vi "libssh2_session_get_timeout.vi"(8 "error in (no error)":errorcluster, 11 "session":T1) -> (0 "error out":errorcluster, 2 "timeout in ms":i32)   [LabVIEW 2017, in "libssh2.lvlib"]
doc: "Get the timeout for blocking functions on a session. A value of zero indicates no timeout."
uses:
  libssh2.lvlib
  Session Refnum.ctl
  Not A Session.vi
  <vilib>/Utility/error.llb/Error Cluster From Error Code.vi
  Global Settings.vi
  Read Session Refnum.vi
  <vilib>/Utility/semaphor.llb/Acquire Semaphore.vi
  <vilib>/Utility/semaphor.llb/Release Semaphore.vi
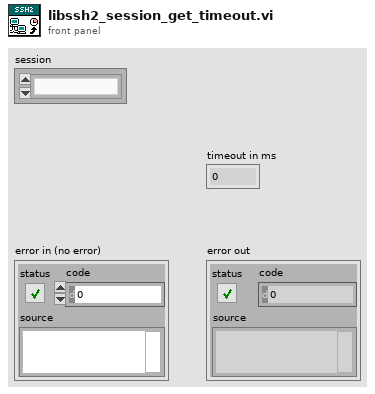
[diagram p1: front panel]
types:
  T1 = typedef "libssh2.lvlib/Session Refnum.ctl" = refnum<k1>
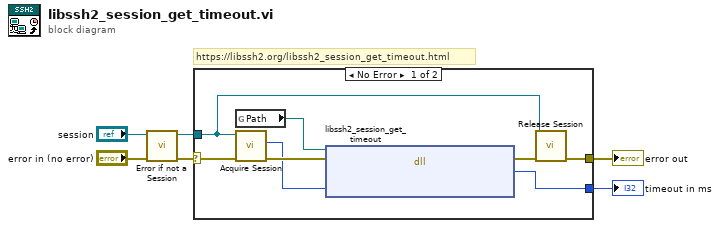
[diagram p0: block diagram]
diagram:
  # "https://libssh2.org/libssh2_session_get_timeout.html"
  n1 = call "Error if not a Session.vi"("error in (no error)"="error in (no error)", "session"="session") -> ("error out"=w4:errorcluster, "session out"=w2:T1)  [unwired: 8 in]
  n2 = case shown="No Error" w4 {
    selector: w4 -> [w13 w15]
    tunnel: [w8 w15] -> w6
    tunnel: w2 -> [w7 _]
    tunnel: [w9 _] -> w1
    frame No Error {
      n3 = global read "Global Settings.vi" "Path"() -> (w10:path)
      n4 = call "Acquire Session.vi"("error in (no error)"=w13, "session"=w7) -> ("error out"=w12:errorcluster, "LIBSSH2_SESSION*"=w11:u64)  [unwired: 7 in, 1 out]
      n5 = dll-call lib="?" fn="libssh2_session_get_timeout"(path in=w10, error in=w12, "session"=w11) -> (error out=w14:errorcluster, "return value"=w9:i32)  [unwired: 2 in, 1 out]
      n6 = call "Release Session.vi"("error in (no error)"=w14, "session"=w7) -> ("error out"=w8:errorcluster)  [unwired: 9 in]
    }
    frame Error {
    }
  }
  "error out" <- w6
  "timeout in ms" <- w1
